vi "isInheritance.vi"(0 "reference":refnum<class "ClassRelationshipEdge.lvclass">, 5 "error in (no error)":errorcluster) -> (14 "reference out":refnum<class "ClassRelationshipEdge.lvclass">, 15 "isInheritance":bool, 16 "isCompAggregation":bool, 18 "isInterfaecImplementing":bool, 19 "error out":errorcluster)   [LabVIEW 2020, in "ClassRelationshipEdge.lvclass"]
uses:
  <resource>/Framework/Providers/Open_GDS/UML/ClassRelationshipEdge_class/ClassRelationshipEdge.lvclass
  C:/Program Files (x86)/National Instruments/LabVIEW 2020/resource/Framework/Providers/Open_GDS/UML/SegmentedLineEdge_class/SegmentedLineEdge.lvclass
  <resource>/Framework/Providers/Open_GDS/UML/ArrowHead_class/ArrowHead.lvclass
  <resource>/Framework/Providers/Open_GDS/UML/LineStyle_class/LineStyle.lvclass
  <resource>/Framework/Providers/Open_GDS/UML/SegmentedLineEdge_class/SegmentedLineEdge.lvclass
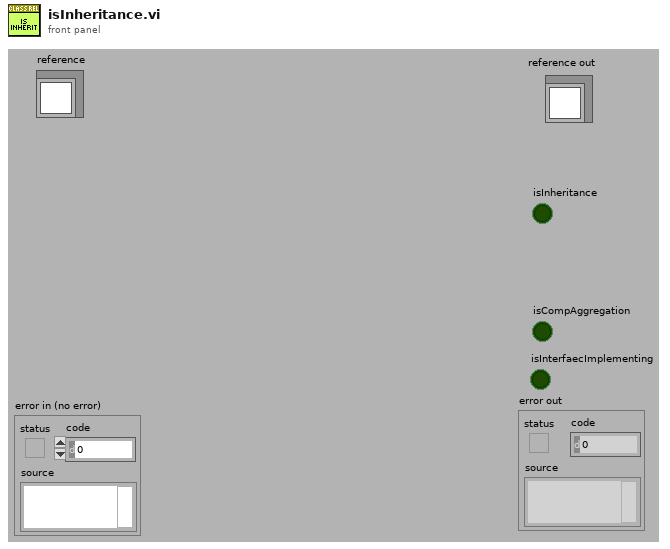
[diagram p1: front panel]
types:
  T1 = typedef "SegmentedLineEdge.lvclass/ObjectAttributes.ctl" = cluster{"lineStyle":refnum<class "LineStyle.lvclass">, "startArrowHead":refnum<class "ArrowHead.lvclass">, "endArrowHead":refnum<class "ArrowHead.lvclass">, "startLabel":string, "midLabel":string, "endLabel":string, "MidLabelOffset":T2, "SplitWire":bool}
  T2 = typedef "Point Point2D.ctl" = cluster{"x":dbl, "y":dbl}
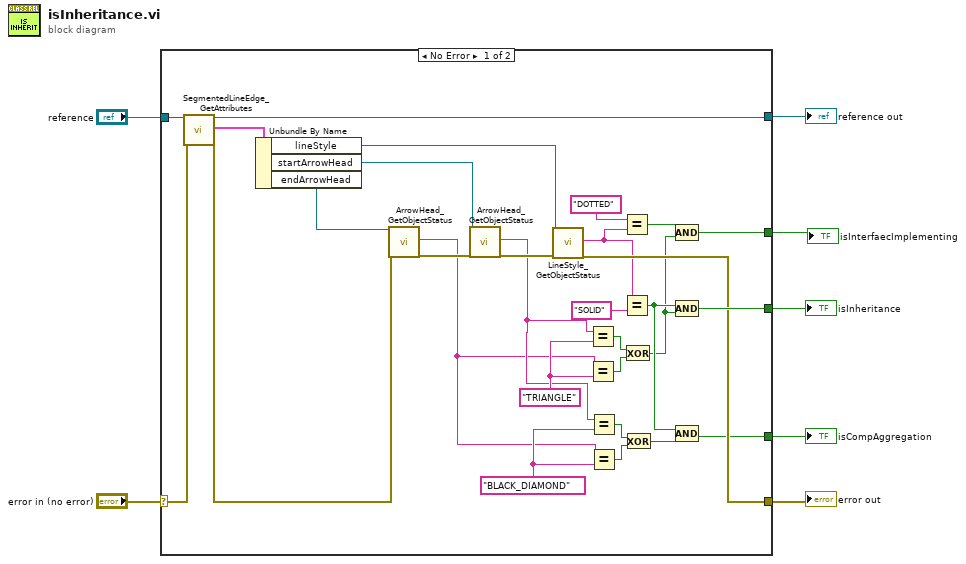
[diagram p0: block diagram]
diagram:
  n1 = case shown="No Error" "error in (no error)" {
    selector: "error in (no error)" -> [w36 w37]
    tunnel: "reference" -> [w35 w38]
    tunnel: [w24 w37] -> w5
    tunnel: [w34 w38] -> w4
    tunnel: [w25 _] -> w2
    tunnel: [w16 _] -> w3
    tunnel: [w8 _] -> w1
    frame No Error {
      w19 = "BLACK_DIAMOND" ("y")
      w30 = "TRIANGLE" ("y")
      n2 = call <resource>:"SegmentedLineEdge_GetAttributes.vi"("reference in"=w35, "error in (no error)"=w36) -> ("reference out"=w34:refnum<class "ClassRelationshipEdge.lvclass">, "Data"=w15:T1, "error out"=w32:errorcluster)  [unwired: 14 in, 1 out]
      n3 = Unbundle By Name(w15) -> ("lineStyle"=w27:refnum<class "LineStyle.lvclass">, "startArrowHead"=w31:refnum<class "ArrowHead.lvclass">, "endArrowHead"=w33:refnum<class "ArrowHead.lvclass">)
      n4 = call <resource>:"ArrowHead_GetObjectStatus.vi"("reference in"=w33, "error in (no error)"=w32) -> ("Object name"=w13:string, "error out"=w29:errorcluster)  [unwired: 1 in, 15 out]
      n5 = call <resource>:"ArrowHead_GetObjectStatus.vi"("reference in"=w31, "error in (no error)"=w29) -> ("Object name"=w14:string, "error out"=w28:errorcluster)  [unwired: 1 in, 15 out]
      n6 = call <resource>:"LineStyle_GetObjectStatus.vi"("reference"=w27, "error in (no error)"=w28) -> ("Type(String)"=w11:string, "error out"=w24:errorcluster)  [unwired: 15 in, 1 out]
      n7 = Equal?(x=w14, y=w30) -> (x = y?=w23:bool)
      n8 = Equal?(x=w13, y=w30) -> (x = y?=w22:bool)
      n9 = Equal?(x=w14, y=w19) -> (x = y?=w20:bool)
      n10 = Equal?(x=w13, y=w19) -> (x = y?=w21:bool)
      n11 = Equal?(x="DOTTED" ("y"), y=w11) -> (x = y?=w9:bool)
      n12 = Equal?(x=w11, y="SOLID") -> (x = y?=w17:bool)
      n13 = Exclusive Or(1:w22, 2:w23) -> (0:w12:bool)
      n14 = Exclusive Or(1:w21, 2:w20) -> (0:w18:bool)
      n15 = Compound Arithmetic op=AND(w9, w12) -> (w8:bool)
      n16 = Compound Arithmetic op=AND(w17, w12) -> (w25:bool)
      n17 = Compound Arithmetic op=AND(w17, w18) -> (w16:bool)
    }
    frame Error {
    }
  }
  "reference out" <- w4
  "error out" <- w5
  "isInheritance" <- w2
  "isCompAggregation" <- w3
  "isInterfaecImplementing" <- w1
